vi "PicoScope2000aExampleRapidBlockBulkOverlapped.vi"() -> ()   [LabVIEW 2010]
uses:
  shared/PicoBuffers.ctl
  <vilib>/Waveform/DWDTOps.llb/DWDT Analog to Digital.vi
  shared/Segment Range.ctl
  shared/Buffer and Transfer Settings.ctl
  shared/Acquisition Settings.ctl
  shared/nSegments.ctl
  PicoScope2000aLib/PicoScope2000aDigitalChannelSettings.ctl
  PicoScope2000aLib/PicoScope2000aAnalogChannelSettings.ctl
panel:
  out "Properties Panel":T1 {"Max Total Capture Time Available (sec)" format="%.3p"; "Sample Frequency" format="%.3p"; "Sample Internal" format="%.3p"; "Max Samples Available" format="%.3p"; "Total Capture Time (sec)" format="%.3p"}
  in  "Trigger Settings":T2={"Trigger Enabled"=FALSE, "Trigger Source"=enum."Channel A", "Trigger Threshold (Volts)"=0.0, "Trigger Direction"=2, "Trigger Delay (samples)"=0, "Auto Trigger Time (ms)"=1000} {"Trigger Direction" items=["Rising"=2, "Falling"=3]}
  in  "Channel A Settings":T3={"Enabled"=TRUE, "Coupling"=1, "Range"=6, "Analogue Offset"=0.0} {"Analogue Offset" format="%#_6p"; "Range" items=["20 mV"=1, "50 mV"=2, "100 mV"=3, "200 mV"=4, "500 mV"=5, "1 V"=6, "2 V"=7, "5 V"=8, "10 V"=9, "20 V"=10]; "Coupling" items=["AC", "DC"]}
  out "Device Info":T4
  out "overflow":i16[](array[numeric]) format="%06b"
  in  "Port 0 Settings":T5={"Enabled"=FALSE, "Logic Level"=9830} {"Logic Level" items=["1.5V TTL"=9830, "2.5V CMOS"=16383]}
  in  "Stop Display":bool
  out "Capture Complete":bool
  in  "Run":bool
  in  "Display Buffer Index":i32
  in  "Segment Range":T6={"fromSegmentIndex"=0, "toSegmentIndex"=9} {"toSegmentIndex" format="%.4p"; "fromSegmentIndex" format="%.4p"}
  in  "nSegments":T7=10 format="%.4p"
  out "error out":errorcluster
  in  "Data file":path=path "PicoScope2000aExampleRapidBlock ChA Data"
  in  "Buffer and Transfer Settings":T8={"startIndex"=0, "Samples"=1000, "Down Sample Ratio"=1, "Down-Sample Mode"=0} {"Down-Sample Mode" items=["RAW none"=2147483648, "None"=0, "Aggregate"=1, "Decimate"=2, "Average"=4]; "Down Sample Ratio" step=1; "Samples" format="%_6p"}
  in  "Acquisition Settings":T9={"preTriggerSamples"=0, "postTriggerSamples"=1000, "timebase"=5} {"postTriggerSamples" format="%_6p"; "preTriggerSamples" format="%_6p"}
  out "Port 0":digitalwaveform(graph)={"t0"=timestamp(0 s since 1904-01-01), "dt"=8e-09, "Y"={"transitions"=[], "data"=[]}}
  in  "stop":bool
  out "Analog Channels":cluster{i32, sgl, "Data":dbl[]}[](graph)
  in  "Serial Number":string
  in  "Use Serial Number":bool
  in  "error in (no error)":errorcluster
  # "Number of\nSegments to Capture"
  # "Bit 0 = ChA"
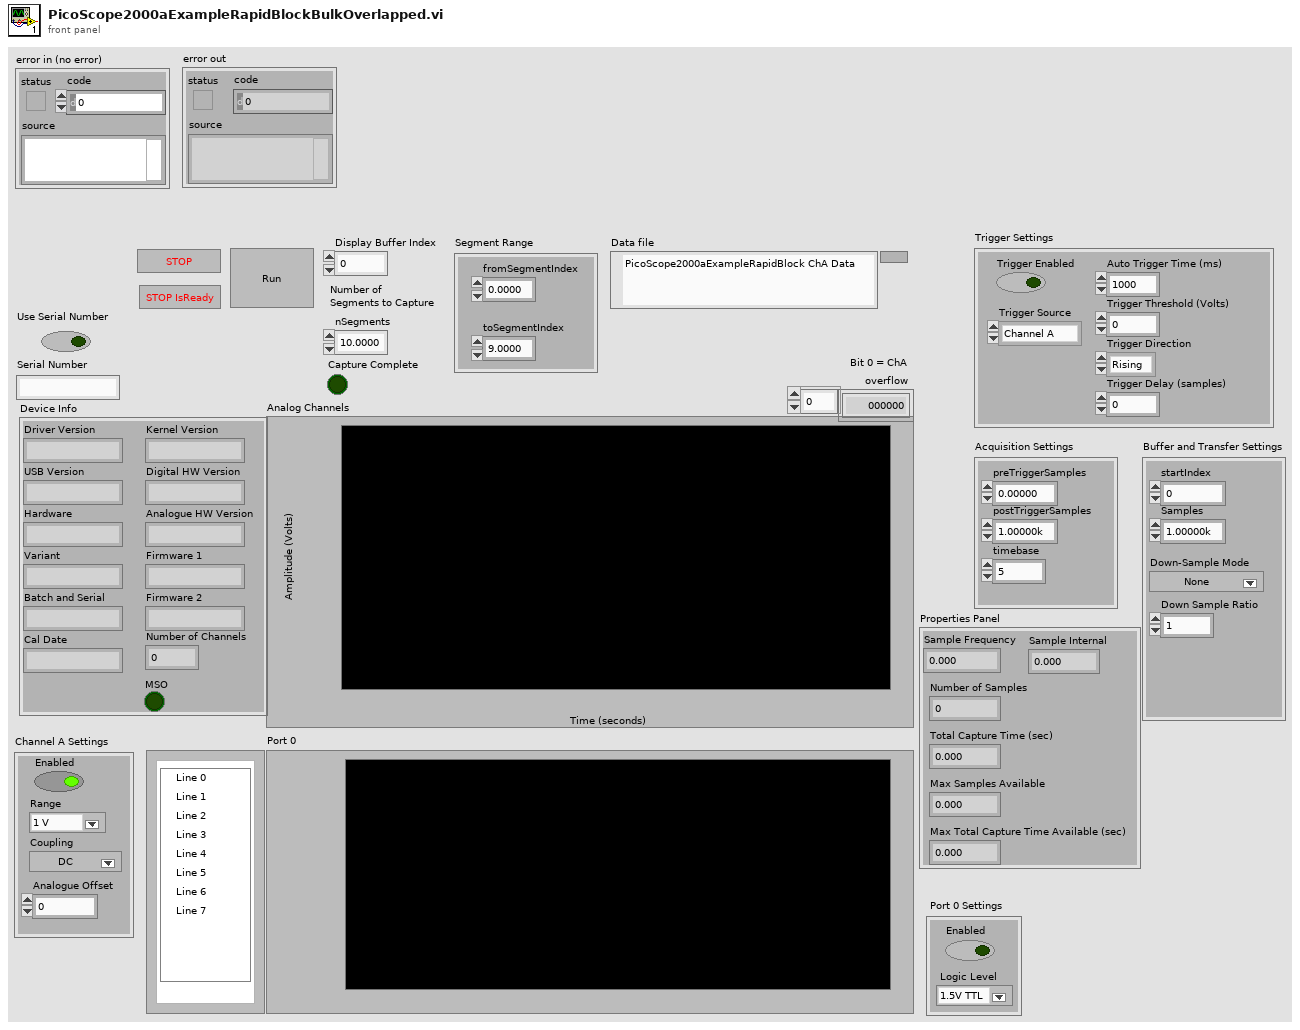
[diagram p1: front panel]
types:
  T1 = cluster{"Sample Frequency":sgl, "Sample Internal":sgl, "Max Samples Available":i32, "Number of Samples":u32, "Total Capture Time (sec) ":sgl, "Max Total Capture Time Available (sec)":sgl}
  T2 = cluster{"Trigger Enabled":bool, "Trigger Source":enum16{"Channel A", "Channel B", "Channel C", "Channel D", "Ext."}, "Trigger Threshold (Volts)":dbl, "Trigger Direction":u16, "Trigger Delay (samples)":u32, "Auto Trigger Time (ms)":i16}
  T3 = typedef "PicoScope2000aAnalogChannelSettings.ctl" = cluster{"Enabled":bool, "Coupling":i16, "Range":u16, "Analogue Offset":sgl}
  T4 = cluster{"Driver Version":string, "USB Version":string, "Hardware":string, "Variant":string, "Batch and Serial":string, "Cal Date":string, "Kernel Version":string, "Digital HW Version":string, "Analogue HW Version":string, "Firmware 1":string, "Firmware 2":string, "MSO":bool, "Number of Channels":i16}
  T5 = typedef "PicoScope2000aDigitalChannelSettings.ctl" = cluster{"Enabled":bool, "Logic Level":i16}
  T6 = typedef "Segment Range.ctl" = cluster{"fromSegmentIndex":u64, "toSegmentIndex":u64}
  T7 = typedef "nSegments.ctl" = u64
  T8 = typedef "Buffer and Transfer Settings.ctl" = cluster{"startIndex":u64, "Samples":u64, "Down Sample Ratio":u64, "Down-Sample Mode":u32}
  T9 = typedef "Acquisition Settings.ctl" = cluster{"preTriggerSamples":u64, "postTriggerSamples":u64, "timebase":u32}
  T10 = enum16{"open", "open or create", "create or replace", "create", "open (read-only)"}
  T11 = typedef "PicoBuffers.ctl" = cluster{"Max Buffer Pointers":u64[][][], "Min Buffer Pointers":u64[][][], "StreamingDataInfo":cluster{"Channel":u32, "Down-Sample Mode":u32, "PICO_DATA_TYPE":enum32{"PICO_INT8_T", "PICO_INT16_T", "PICO_INT32_T", "PICO_UINT32_T", "PICO_INT64_T", ""}, "Samples":i32, "bufferIndex":u64, "startIndex":i32, "overflow":i16}[][]}
  T12 = cluster{"Channel A Buffer":i16[], "Channel B Buffer":i16[], "Channel C Buffer":i16[], "Channel D Buffer":i16[], "Channel E Buffer":i16[], "Channel F Buffer":i16[], "Channel G Buffer":i16[], "Channel H Buffer":i16[], "Port 0 Buffer":i16[], "Port 1 Buffer":i16[]}[]
  T13 = cluster{"Channel A Buffer":i16[], "Channel B Buffer":i16[], "Channel C Buffer":i16[], "Channel D Buffer":i16[], "Channel E Buffer":i16[], "Channel F Buffer":i16[], "Channel G Buffer":i16[], "Channel H Buffer":i16[], "Port 0 Buffer":i16[], "Port 1 Buffer":i16[]}
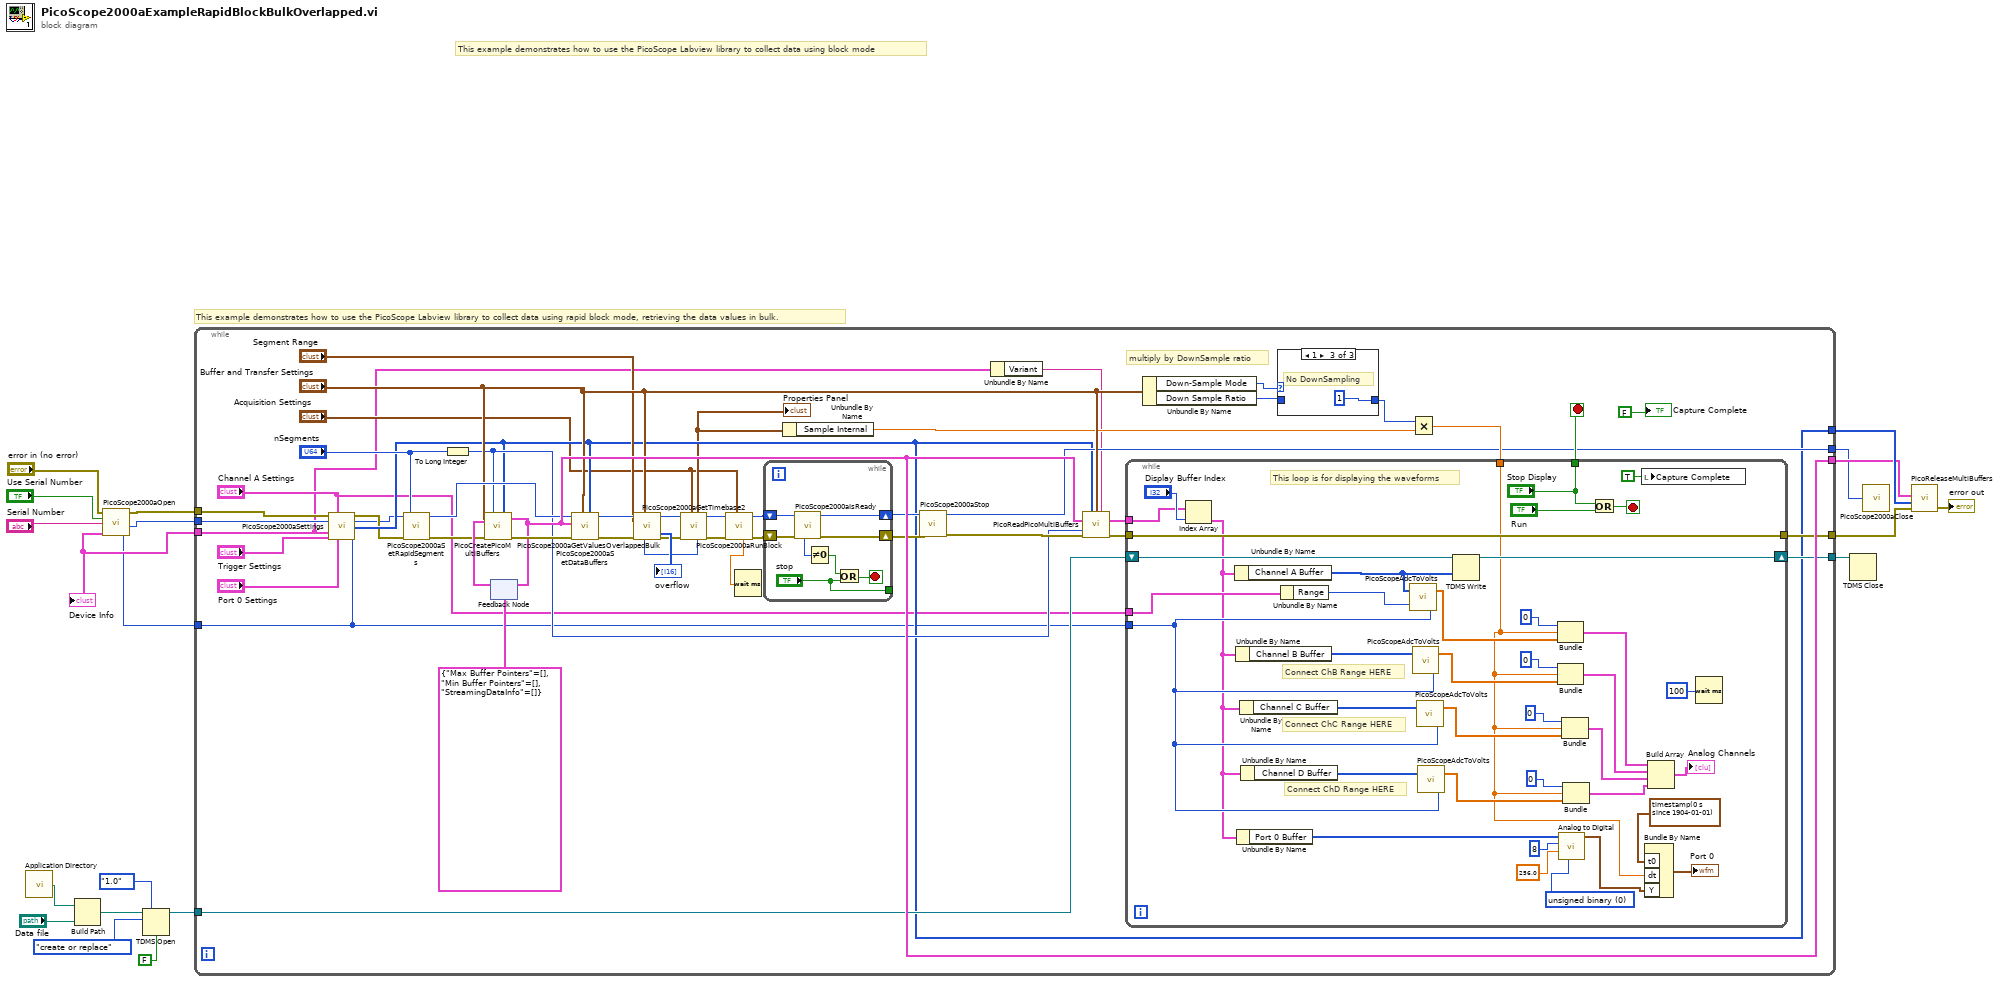
[diagram p0: block diagram]
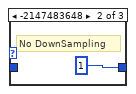
[diagram p3: hidden frame]
diagram:
  # "This example demonstrates how to use the PicoScope Labview library to collect data using rapid block mode, retrieving the data values in bulk."
  # "This example demonstrates how to use the PicoScope Labview library to collect data using block mode"
  n1 = call <vilib>:"Application Directory.vi"() -> ("Application Directory"=w11:path)
  n2 = Build Path(base path=w11, name or relative path="Data file") -> (appended path=w12:path)
  n3 = call "PicoScope2000aOpen.vi"("Serial Number"="Serial Number", "Use Serial Number"="Use Serial Number", "error in (no error)"="error in (no error)") -> ("Max Adc value"=w1:i16, "handle"=w20:i16, "error out"=w3:errorcluster, "Device Info"=w4:T4)  [unwired: 1 in]
  "Device Info" <- w4
  n4 = TDMS Open(6:FALSE ("disable buffering? (T)"), 7:enum16{"1.0", "2.0"}."1.0" ("file format version (2.0)"), 10:T10."create or replace" ("operation (0:open)"), 11:w12) -> (3:w9:refnum<k34>)  [unwired: 2 in, 1 out]
  n5 = while {
    tunnel: w20 -> [w36]
    tunnel: w1 -> [w22]
    tunnel: [w46] -> w17
    tunnel: [w38] -> w19
    tunnel: [w67] -> w18
    tunnel: [w66] -> w10
    tunnel: w9 -> [w65]
    tunnel: w4 -> [w21]
    tunnel: w3 -> [w35]
    tunnel: [w44] -> w2
    stop <- w51 stop-if-true
    # "multiply by DownSample ratio"
    n6 = call "PicoScope2000aSettings.vi"("error in"=w35, "Channel A Settings"="Channel A Settings", "handle in"=w36, "Trigger Settings"="Trigger Settings", "Port 0 Settings"="Port 0 Settings", "Device Info"=w21, "Max_adc"=w22) -> ("error out"=w34:errorcluster, "handle out"=w33:i16, "Enabled Array"=w38:i16[])  [unwired: 6 in]
    n7 = call "PicoScope2000aSetRapidSegments.vi"("nSegments"="nSegments", "error in (no error)"=w34, "handle in"=w33) -> ("error out"=w64:errorcluster, "handle out"=w63:i16)  [unwired: 6 in, 1 out]
    n8 = To Long Integer(number="nSegments") -> (32bit integer=w43:i32)
    n9 = feedback #1(T11 {"Max Buffer Pointers"=[], "Min Buffer Pointers"=[], "StreamingDataInfo"=[]} ("Data Pointers")) -> (w69:T11)
    n10 = call "PicoCreatePicoMultiBuffers.vi"("Number of Buffers"=w43, "Buffer and Transfer Settings"="Buffer and Transfer Settings", "enabled array"=w38, "Data Pointers In"=w69, "error in (no error)"=w64) -> ("Data Pointers"=w67:T11, "error out"=w68:errorcluster)  [unwired: 9 in]
    n11 = feedback-in #1(w67) -> ()
    n12 = call "PicoScope2000aSetDataBuffers.vi"("enabled array"=w38, "Buffer and Transfer Settings"="Buffer and Transfer Settings", "error in (no error)"=w68, "Data Pointers In"=w67, "handle in"=w63) -> ("error out"=w62:errorcluster, "handle out"=w61:i16)  [unwired: 5 in]
    n13 = call "PicoScope2000aGetValuesOverlappedBulk.vi"("Segment Range"="Segment Range", "Buffer and Transfer Settings"="Buffer and Transfer Settings", "error in (no error)"=w62, "handle in"=w61) -> ("error out"=w28:errorcluster, "handle out"=w25:i16, "overflow"=→"overflow":i16[], "noOfSamples"=w23:u64)  [unwired: 4 in]
    n14 = call "PicoScope2000aGetTimebase2.vi"("Number of Samples"=w23, "Acquisition Settings"="Acquisition Settings", "error in (no error)"=w28, "handle in"=w25) -> ("error out"=w27:errorcluster, "handle out"=w26:i16, "Properties Panel"=w29:T1)  [unwired: 5 in]
    "Properties Panel" <- w29
    n15 = call "PicoScope2000aRunBlock.vi"("Acquisition Settings"="Acquisition Settings", "error in (no error)"=w27, "handle in"=w26) -> ("error out"=w54:errorcluster, "handle out"=w53:i16, "timeIndisposedMs"=w30:dbl)  [unwired: 5 in, 1 out]
    n16 = Wait (ms)(milliseconds to wait=w30) -> ()  [unwired: 1 out]
    n17 = while {
      shift-right: [w116] -> w48
      shift-left: w54 -> [w117]
      shift-right: [w115] -> w45
      shift-left: w53 -> [w114]
      tunnel: ["stop"] -> _
      stop <- w111 stop-if-true
      n18 = call "PicoScope2000aIsReady.vi"("error in (no error)"=w117, "handle in"=w114) -> ("error out"=w116:errorcluster, "handle out"=w115:i16, "ready"=w113:i16)  [unwired: 7 in]
      n19 = Not Equal To 0?(x=w113) -> (x != 0?=w112:bool)
      n20 = Or(x=w112, y="stop") -> (x .or. y?=w111:bool)
    }
    n21 = Unbundle By Name(w29) -> ("Sample Internal"=w40:sgl)
    n22 = call "PicoScope2000aStop.vi"("error in (no error)"=w48, "handle in"=w45) -> ("error out"=w47:errorcluster, "handle out"=w46:i16)  [unwired: 8 in]
    n23 = Unbundle By Name(w21) -> ("Variant"=w39:string)
    n24 = call "PicoReadPicoMultiBuffers.vi"("enabled array"=w38, "Buffer and Transfer Settings"="Buffer and Transfer Settings", "Variant"=w39, "Data Pointers"=w67, "No of Buffers"=w43, "error in (no error)"=w47) -> ("MultiBuffers (Max or non-aggregated)"=w59:T12, "error out"=w52:errorcluster)  [unwired: 7 in, 1 out]
    n25 = Unbundle By Name("Buffer and Transfer Settings") -> ("Down-Sample Mode"=w57:u32, "Down Sample Ratio"=w58:u64)
    n26 = case shown="1" w57 {
      tunnel: [w118 u64 1 ("Down Sample Ratio") u64 1 ("Down Sample Ratio")] -> w55
      tunnel: w58 -> [w118 _ _]
      frame Default {
      }
      frame -2147483648 {
        # "No DownSampling"
      }
      frame 1 {
        # "No DownSampling"
      }
    }
    n27 = Multiply(x=w55, y=w40) -> (x*y=w56:sgl)
    n28 = while {
      tunnel: w22 -> [w72]
      tunnel: "Channel A Settings" -> [w109]
      tunnel: w59 -> [w82]
      tunnel: w56 -> [w74]
      shift-right: [w108] -> w66
      shift-left: w65 -> [w107]
      tunnel: [w88] -> w44
      tunnel: w52 -> [w88]
      tunnel: ["Stop Display"] -> w51
      stop <- w85 stop-if-true
      w97 = u16 0 items=["unsigned binary", "offset binary", "2's complement"] ("data format (offset binary)")
      # "This loop is for displaying the waveforms"
      # "Connect ChB Range HERE"
      # "Connect ChD Range HERE"
      # "Connect ChC Range HERE"
      n29 = Index Array(array=w82, index="Display Buffer Index") -> (element=w71:T13)
      n30 = Unbundle By Name(w71) -> ("Channel A Buffer"=w90:i16[])
      n31 = Unbundle By Name(w71) -> ("Channel B Buffer"=w103:i16[])
      n32 = Unbundle By Name(w71) -> ("Port 0 Buffer"=w95:i16[])
      n33 = Unbundle By Name(w71) -> ("Channel C Buffer"=w80:i16[])
      n34 = Unbundle By Name(w71) -> ("Channel D Buffer"=w76:i16[])
      n35 = Unbundle By Name(w109) -> ("Range"=w105:u16)
      n36 = call "PicoScopeAdcToVolts.vi"("Max_adc"=w72, "Range Index"=w105, "Data"=w90) -> ("Data"=w91:dbl[])
      n37 = call "PicoScopeAdcToVolts.vi"("Max_adc"=w72, "Data"=w103) -> ("Data"=w102:dbl[])  [unwired: 1 in]
      n38 = call "PicoScopeAdcToVolts.vi"("Max_adc"=w72, "Data"=w80) -> ("Data"=w79:dbl[])  [unwired: 1 in]
      n39 = call "PicoScopeAdcToVolts.vi"("Max_adc"=w72, "Data"=w76) -> ("Data"=w75:dbl[])  [unwired: 1 in]
      n40 = TDMS Write(0:w107, 9:w90) -> (4:w108:refnum<k34>)  [unwired: 4 in, 3 out]
      n41 = Bundle(0, w74, "Data"=w91) -> (w101:cluster{i32, sgl, "Data":dbl[]})  [unwired: 1 in]
      n42 = Bundle(0, w74, "Data"=w102) -> (w100:cluster{i32, sgl, "Data":dbl[]})  [unwired: 1 in]
      n43 = call-poly <vilib>:"Analog to Digital.vi"("data format (offset binary)"=w97, "full-scale range (pk-pk)"=256.0, "resolution (16 bit)"=8, "analog waveform"=w95) -> ("digital waveform"=w92:digitalwaveform)  [unwired: 4 in, 3 out]
      n44 = Bundle(0, w74, "Data"=w79) -> (w78:cluster{i32, sgl, "Data":dbl[]})  [unwired: 1 in]
      n45 = Bundle(0, w74, "Data"=w75) -> (w73:cluster{i32, sgl, "Data":dbl[]})  [unwired: 1 in]
      n46 = Or(x="Stop Display", y="Run") -> (x .or. y?=w85:bool)
      n47 = local write "Capture Complete"(TRUE ("Capture Complete")) -> ()
      n48 = Bundle By Name("t0"=timestamp(0 s since 1904-01-01), "dt"=w74, "Y"=w92) -> (→"Port 0":digitalwaveform)  [unwired: 1 in]
      n49 = Build Array(w101, w100, w78, w73) -> (→"Analog Channels":cluster{i32, sgl, "Data":dbl[]}[])
      n50 = Wait (ms)(milliseconds to wait=u32 100) -> ()  [unwired: 1 out]
    }
    "Capture Complete" <- FALSE ("Capture Complete")
  }
  n51 = TDMS Close(11:w10) -> ()  [unwired: 1 in, 2 out]
  n52 = call "PicoScope2000aClose.vi"("handle"=w17) -> ()
  n53 = call "PicoReleaseMultiBuffers.vi"("error in (no error)"=w2, "Enabled array"=w19, "Data Pointers"=w18) -> ("error out"=→"error out":errorcluster)  [unwired: 8 in]
